vi "K_S30 F73 read Value.vi"(7 "VISA resource":refnum<visa-resource-name>, 8 "error in":errorcluster, 10 "Channel":enum16{"CH0", "P1", "P2", "T", "TOB1", "TOB2"}(ring), 11 "Address":u8=250) -> (0 "error out":errorcluster, 2 "Status":u8 format="%.0b", 3 "Value":sgl format="%.6e")   [LabVIEW 2022 SP3]
panel:
  # "Function 73: Read Value of a Channel\nV1.0, b.v."
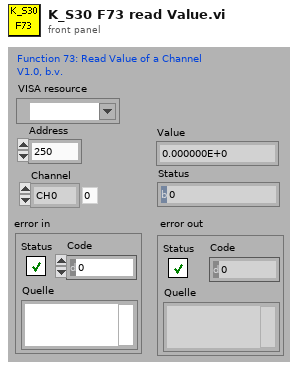
[diagram p1: front panel]
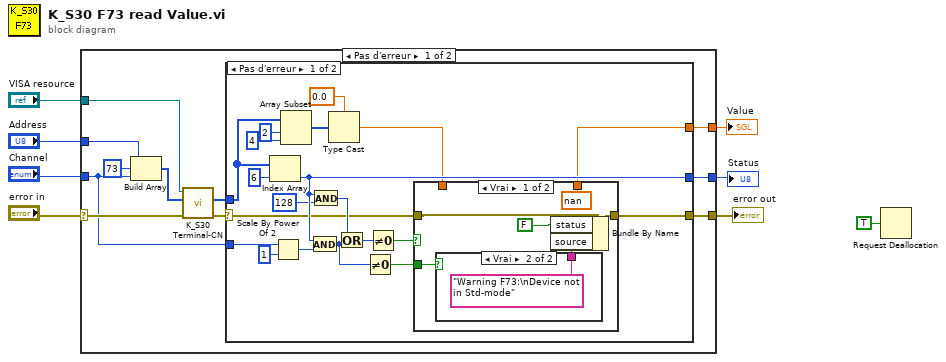
[diagram p0: block diagram]
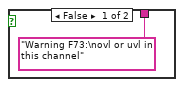
[diagram p2: hidden frame]
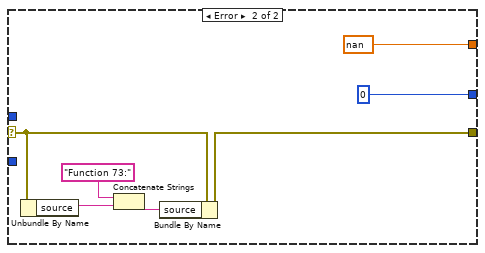
[diagram p4: hidden frame]
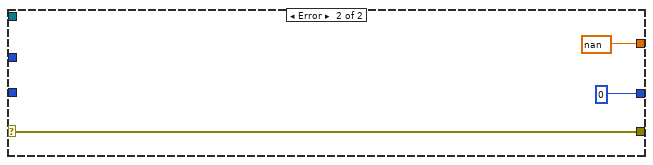
[diagram p5: hidden frame]
diagram:
  n1 = case shown="Pas d'erreur" "error in" {
    selector: "error in" -> [w16 w59]
    tunnel: "Address" -> [w19 _]
    tunnel: [w14 w59] -> w6
    tunnel: "Channel" -> [w12 _]
    tunnel: [w11 u8 0] -> w4
    tunnel: [w10 sgl nan] -> w3
    tunnel: "VISA resource" -> [w9 _]
    frame No Error {
      n2 = Build Array(w19, u8 73 ("Element"), w12) -> (w17:u16[])
      n3 = call "K_S30 Terminal-CN.vi"("error in"=w16, "request"=w17, "VISA resource"=w9) -> ("error out"=w15:errorcluster, "response"=w13:u8[])  [unwired: 7 in]
      n4 = case shown="Pas d'erreur" w15 {
        selector: w15 -> [w27 w56]
        tunnel: [w26 w54] -> w14
        tunnel: w13 -> [w35 _]
        tunnel: [w22 sgl nan] -> w10
        tunnel: [w31 u8 0] -> w11
        tunnel: w12 -> [w32 _]
        frame No Error {
          n5 = Index Array(array=w35, index=6 ("Index")) -> (element=w31:u8)
          n6 = Scale By Power Of 2(n=w32, x=u8 1) -> (x*2^n=w29:u8)
          n7 = Array Subset(array=w35, index=2 ("Index"), length=4 ("Länge")) -> (w36:u8[])
          n8 = And(x=w31, y=w29) -> (x .and. y?=w25:u8)
          n9 = And(x=w31, y=u8 128) -> (x .and. y?=w28:u8)
          n10 = Type Cast(type=sgl 0.0, x=w36) -> (*(type *) &x=w23:sgl)
          n11 = Or(x=w28, y=w25) -> (x .or. y?=w21:u8)
          n12 = Not Equal To 0?(x=w25) -> (x != 0?=w24:bool)
          n13 = Not Equal To 0?(x=w21) -> (x != 0?=w20:bool)
          n14 = case shown="Vrai" w20 {
            tunnel: w27 -> [w44 w49]
            tunnel: [w43 w49] -> w26
            tunnel: w24 -> [w45 _]
            tunnel: w23 -> [_ w48]
            tunnel: [nan w48] -> w22
            frame True {
              n15 = case shown="Vrai" w45 {
                tunnel: ["Warning F73:\novl or uvl in this channel" "Warning F73:\nDevice not in Std-mode"] -> w42
                frame False {
                }
                frame True {
                }
              }
              n16 = Bundle By Name(cluster=w44, "status"=FALSE, "source"=w42) -> (w43:errorcluster)
            }
            frame False {
            }
          }
        }
        frame Error {
          n17 = Unbundle By Name(w56) -> ("source"=w52:string)
          n18 = Concatenate Strings("Function 73:" ("String"), w52) -> (w55:string)
          n19 = Bundle By Name(cluster=w56, "source"=w55) -> (w54:errorcluster)
        }
      }
    }
    frame Error {
    }
  }
  "error out" <- w6
  "Status" <- w4
  "Value" <- w3
  n20 = Request Deallocation(TRUE ("flag")) -> ()
